vi "Buffer VI Path by Type.vi"(10 "Repeated":bool, 11 "Proto Type":T1) -> (2 "Decode":path, 3 "Encode":path)   [LabVIEW 2020, in "LV-Proto.lvlib"]
uses:
  LV-Proto.lvlib
  Proto Type.ctl
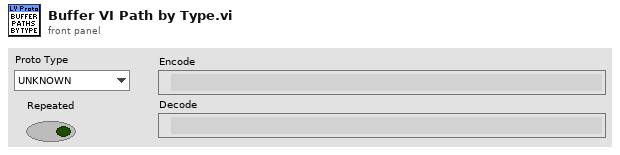
[diagram p1: front panel]
types:
  T1 = typedef "LV-Proto.lvlib/Proto Type.ctl" = enum16{"UNKNOWN", "double", "float", "int32", "int64", "uint32", "uint64", "sint32", "sint64", "fixed32", "fixed64", "sfixed32", "sfixed64", "bool", "string", "bytes", "enum", "map", "message"}
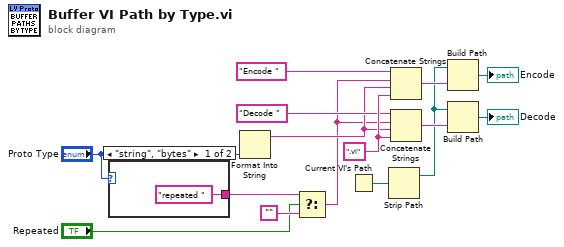
[diagram p0: block diagram]
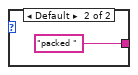
[diagram p2: hidden frame]
diagram:
  w14 = ".vi" ("string")
  n1 = case shown="\"string\", \"bytes\"" "Proto Type" {
    tunnel: ["repeated " "packed "] -> w1
    frame "string", "bytes" {
    }
    frame Default {
    }
  }
  n2 = Format Into String("Proto Type") -> (resulting string=w11:string)  [unwired: 3 in, 1 out]
  n3 = Select(t=w1, s="Repeated", f="") -> (s? t:f=w3:string)
  n4 = Current VI's Path() -> (path=w15:path)
  n5 = Strip Path(path=w15) -> (stripped path=w8:path)  [unwired: 1 out]
  n6 = Concatenate Strings("Encode ", w3, w11, w14) -> (w10:string)
  n7 = Concatenate Strings("Decode ", w3, w11, w14) -> (w9:string)
  n8 = Build Path(base path=w8, name or relative path=w10) -> (appended path=→"Encode":path)
  n9 = Build Path(base path=w8, name or relative path=w9) -> (appended path=→"Decode":path)
